vi "test_toml_reader.vi"(8 "error in (no error)":errorcluster, 11 "dragon_file_path":path=path "C:/Projects/toml-edit-labview/lv_src/test.toml") -> ()   [LabVIEW 2020]
uses:
  Doc/Doc.lvclass
  Table/Table.lvclass
  Item/Item.lvclass
  Value/Value.lvclass
  InlineTable/InlineTable.lvclass
  Item/type--enum.ctl
  Value/value_type--enum.ctl
panel:
  out "Contains Item":bool[](array[boolean])
  out "item_types":T1[](array[typedef])
  out "values":string[](array[string])
  out "item_names 2":string[](array[string])
  out "inline_table_item_names":string[](array[string])
  out "value_types":T2[](array[typedef])
  out "item_types":T1[](array[typedef])
  out "item_names":string[](array[string])
  out "value_strings":string[](array[string])
  out "item_names":string[](array[string])
  out "item_types":T1[](array[typedef])
  out "integer_value":i64
  out "string_value":string
  out "value_type":T2
  out "item_type":T1
  out "tables":string[](array[string])
  out "error out":errorcluster
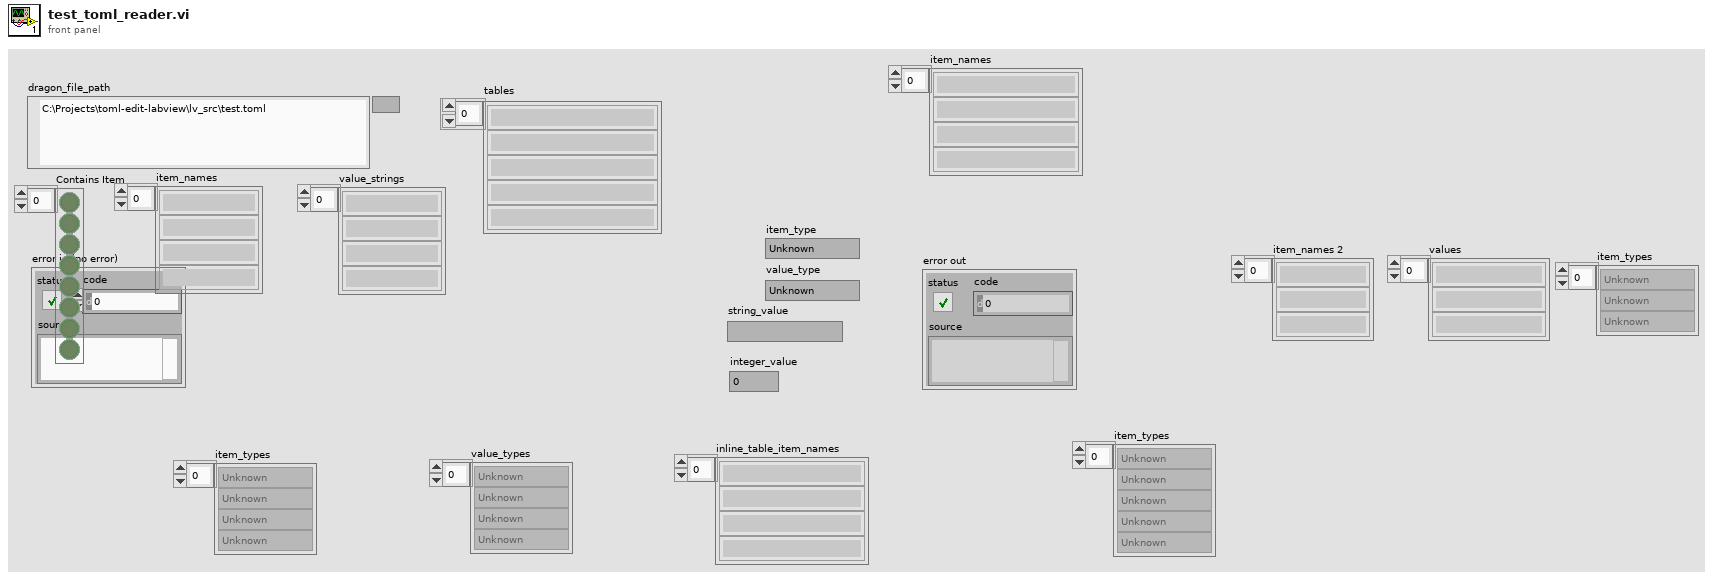
[diagram p1: front panel]
types:
  T1 = typedef "toml_edit.lvlib/Item.lvclass/type--enum.ctl" = enum16{"Unknown", "None", "Value", "ArrayOfTables", "Table"}
  T2 = typedef "toml_edit.lvlib/Value.lvclass/value_type--enum.ctl" = enum16{"Unknown", "String", "Integer", "Float", "Boolean", "Datetime", "Array", "InlineTable"}
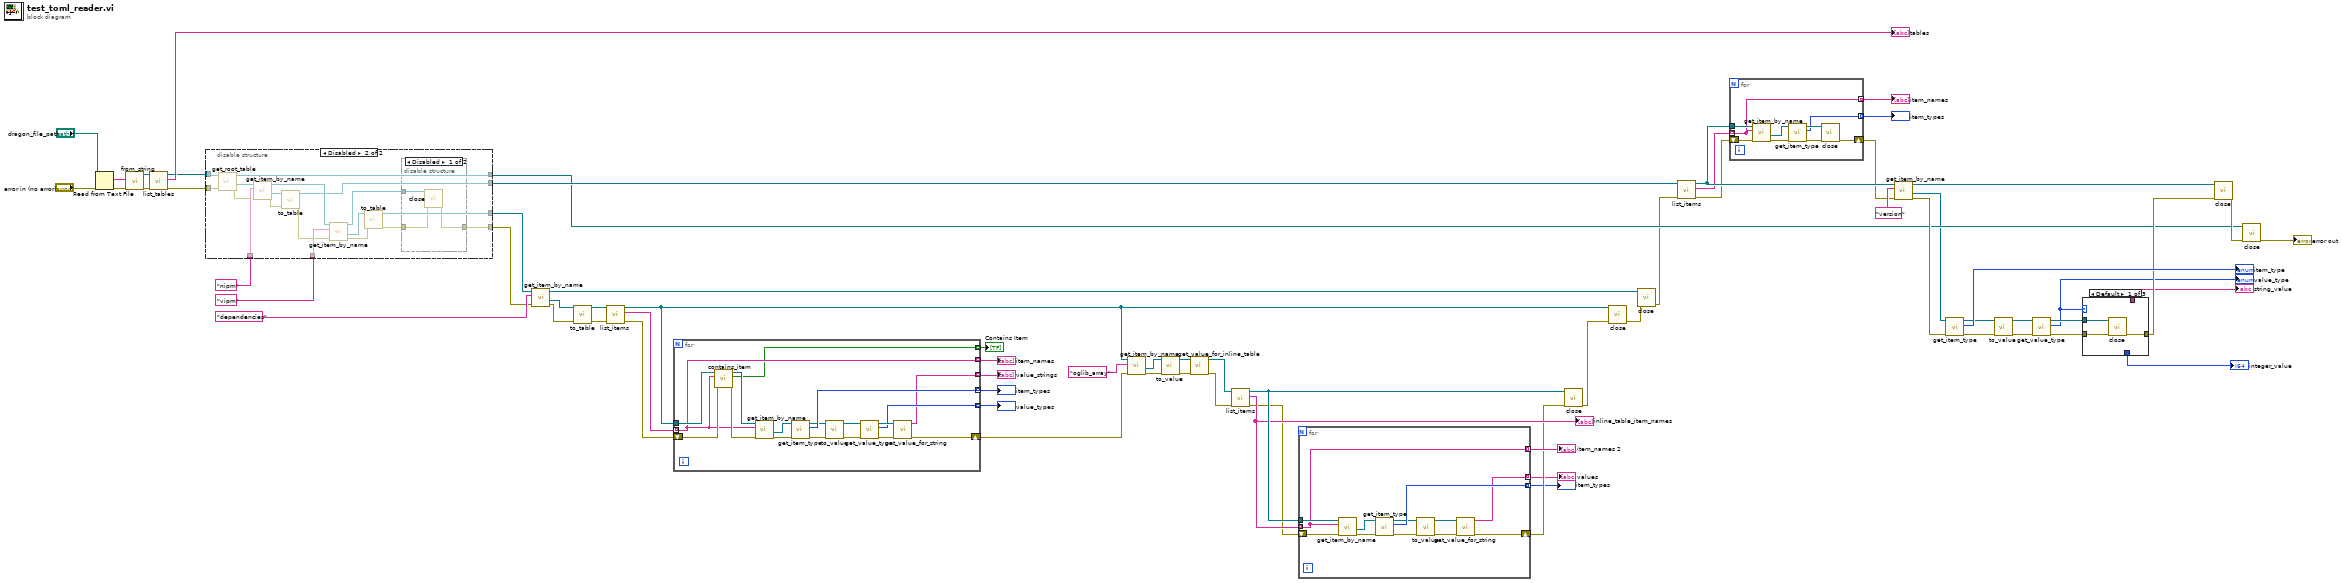
[diagram p0: block diagram]
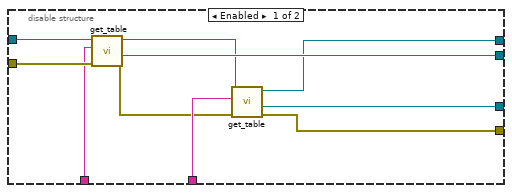
[diagram p2: hidden frame]
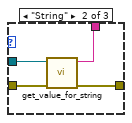
[diagram p4: hidden frame]
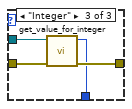
[diagram p5: hidden frame]
diagram:
  n1 = Read from Text File(file (use dialog)="dragon_file_path", error in="error in (no error)") -> (text=w67:string, error out=w66:errorcluster)  [unwired: 2 in, 2 out]
  n2 = call "from_string.vi"("error in (no error)"=w66, "toml"=w67) -> ("error out"=w64:errorcluster, "Doc out"=w65:refnum<class "Doc.lvclass">)  [unwired: 8 in]
  n3 = call "list_tables.vi"("error in (no error)"=w64, "Doc in"=w65) -> ("error out"=w61:errorcluster, "table_names"=→"tables":string[], "Doc out"=w62:refnum<class "Doc.lvclass">)  [unwired: 7 in]
  n4 = disable-structure shown="Disabled" {
    disable-tunnel: w62 -> [w80 w97]
    disable-tunnel: w61 -> [w79 w98]
    disable-tunnel: "nipm" ("table_name") -> [w78 w94]
    disable-tunnel: [w77 w90] -> w39
    disable-tunnel: [w75 w95] -> w38
    disable-tunnel: "vipm" ("table_name") -> [w74 w93]
    disable-tunnel: [w73 w88] -> w36
    disable-tunnel: [w72 w81] -> w19
    frame Enabled {
      n5 = call "get_table.vi"("error in (no error)"=w79, "table_name"=w78, "Doc in"=w80) -> ("error out"=w71:errorcluster, "Table"=w77:refnum<class "Table.lvclass">, "Doc out"=w76:refnum<class "Doc.lvclass">)  [unwired: 5 in, 1 out]
      n6 = call "get_table.vi"("error in (no error)"=w71, "table_name"=w74, "Doc in"=w76) -> ("error out"=w72:errorcluster, "Table"=w73:refnum<class "Table.lvclass">, "Doc out"=w75:refnum<class "Doc.lvclass">)  [unwired: 5 in, 1 out]
    }
    frame Disabled {
      n7 = call "get_root_table.vi"("error in (no error)"=w98, "Doc in"=w97) -> ("error out"=w84:errorcluster, "Table"=w96:refnum<class "Table.lvclass">, "Doc out"=w95:refnum<class "Doc.lvclass">)  [unwired: 7 in]
      n8 = call "get_item_by_name.vi"("error in (no error)"=w84, "item_name"=w94, "Table in"=w96) -> ("error out"=w85:errorcluster, "Item"=w91:refnum<class "Item.lvclass">, "Table out"=w92:refnum<class "Table.lvclass">)  [unwired: 4 in, 2 out]
      n9 = call "to_table.vi"("error in (no error)"=w85, "Item in"=w91) -> ("error out"=w86:errorcluster, "Table"=w90:refnum<class "Table.lvclass">)  [unwired: 8 in]
      n10 = call "get_item_by_name.vi"("error in (no error)"=w86, "item_name"=w93, "Table in"=w92) -> ("error out"=w87:errorcluster, "Item"=w89:refnum<class "Item.lvclass">, "Table out"=w83:refnum<class "Table.lvclass">)  [unwired: 4 in, 2 out]
      n11 = call "to_table.vi"("error in (no error)"=w87, "Item in"=w89) -> ("error out"=w82:errorcluster, "Table"=w88:refnum<class "Table.lvclass">)  [unwired: 8 in]
      n12 = disable-structure shown="Disabled" {
        disable-tunnel: w83 -> [w101 _]
        disable-tunnel: w82 -> [w100 w102]
        disable-tunnel: [w99 w102] -> w81
        frame Disabled {
          n13 = call "close.vi"("error in (no error)"=w100, "Table in"=w101) -> ("error out"=w99:errorcluster)  [unwired: 9 in]
        }
        frame Enabled {
        }
      }
    }
  }
  n14 = call "get_item_by_name.vi"("error in (no error)"=w19, "item_name"="dependencies" ("table_name"), "Table in"=w36) -> ("error out"=w33:errorcluster, "Item"=w18:refnum<class "Item.lvclass">, "Table out"=w31:refnum<class "Table.lvclass">)  [unwired: 4 in, 2 out]
  n15 = call "to_table.vi"("error in (no error)"=w33, "Item in"=w18) -> ("error out"=w34:errorcluster, "Table"=w21:refnum<class "Table.lvclass">)  [unwired: 8 in]
  n16 = call "list_items.vi"("error in (no error)"=w34, "Table in"=w21) -> ("error out"=w28:errorcluster, "items"=w29:string[], "Table out"=w23:refnum<class "Table.lvclass">)  [unwired: 7 in]
  n17 = for {
    tunnel: w23 -> [w108]
    tunnel: w29 -> [w105] mode=indexing
    shift-right: [w116] -> w22
    shift-left: w28 -> [w107]
    tunnel: [w119] -> w25 mode=indexing
    tunnel: [w105] -> w26 mode=indexing
    tunnel: [w103] -> w27 mode=indexing
    tunnel: [w112] -> w24 mode=indexing
    tunnel: [w104] -> w2 mode=indexing
    n18 = call "contains_item.vi"("error in (no error)"=w107, "item_name"=w105, "Table in"=w108) -> ("error out"=w106:errorcluster, "contains_item"=w104:bool, "Table out"=w109:refnum<class "Table.lvclass">)  [unwired: 6 in]
    n19 = call "get_item_by_name.vi"("error in (no error)"=w106, "item_name"=w105, "Table in"=w109) -> ("error out"=w120:errorcluster, "Item"=w110:refnum<class "Item.lvclass">)  [unwired: 4 in, 3 out]
    n20 = call "get_item_type.vi"("error in (no error)"=w120, "Item in"=w110) -> ("error out"=w117:errorcluster, "item_type"=w119:T1, "Item out"=w118:refnum<class "Item.lvclass">)  [unwired: 7 in]
    n21 = call "to_value.vi"("error in (no error)"=w117, "Item in"=w118) -> ("error out"=w114:errorcluster, "Value out"=w111:refnum<class "Value.lvclass">)  [unwired: 8 in]
    n22 = call "get_value_type.vi"("error in (no error)"=w114, "Value in"=w111) -> ("error out"=w113:errorcluster, "value_type"=w112:T2, "Value out"=w115:refnum<class "Value.lvclass">)  [unwired: 7 in]
    n23 = call "get_value_for_string.vi"("error in (no error)"=w113, "Value in"=w115) -> ("error out"=w116:errorcluster, "string_value"=w103:string)  [unwired: 8 in]
  }
  "value_strings" <- w27
  "item_names" <- w26
  "item_types" <- w25
  "value_types" <- w24
  "Contains Item" <- w2
  n24 = call "get_item_by_name.vi"("error in (no error)"=w22, "item_name"="oglib_array", "Table in"=w23) -> ("error out"=w15:errorcluster, "Item"=w3:refnum<class "Item.lvclass">)  [unwired: 4 in, 3 out]
  n25 = call "to_value.vi"("error in (no error)"=w15, "Item in"=w3) -> ("error out"=w14:errorcluster, "Value out"=w13:refnum<class "Value.lvclass">)  [unwired: 8 in]
  n26 = call "get_value_for_inline_table.vi"("error in (no error)"=w14, "Value in"=w13) -> ("error out"=w12:errorcluster, "InlineTable out"=w1:refnum<class "InlineTable.lvclass">)  [unwired: 8 in]
  n27 = call "list_items.vi"("error in (no error)"=w12, "Table in"=w1) -> ("error out"=w7:errorcluster, "items"=w8:string[], "Table out"=w9:refnum<class "InlineTable.lvclass">)  [unwired: 7 in]
  "inline_table_item_names" <- w8
  n28 = for {
    tunnel: w9 -> [w132]
    tunnel: w8 -> [w130] mode=indexing
    shift-right: [w128] -> w6
    shift-left: w7 -> [w131]
    tunnel: [w130] -> w10 mode=indexing
    tunnel: [w121] -> w5 mode=indexing
    tunnel: [w129] -> w4 mode=indexing
    n29 = call "get_item_by_name.vi"("error in (no error)"=w131, "key_name"=w130, "Table in"=w132) -> ("error out"=w127:errorcluster, "Item"=w122:refnum<class "Item.lvclass">)  [unwired: 6 in, 1 out]
    n30 = call "get_item_type.vi"("error in (no error)"=w127, "Item in"=w122) -> ("error out"=w126:errorcluster, "item_type"=w129:T1, "Item out"=w124:refnum<class "Item.lvclass">)  [unwired: 7 in]
    n31 = call "to_value.vi"("error in (no error)"=w126, "Item in"=w124) -> ("error out"=w125:errorcluster, "Value out"=w123:refnum<class "Value.lvclass">)  [unwired: 8 in]
    n32 = call "get_value_for_string.vi"("error in (no error)"=w125, "Value in"=w123) -> ("error out"=w128:errorcluster, "string_value"=w121:string)  [unwired: 8 in]
  }
  "item_names 2" <- w10
  "values" <- w5
  "item_types" <- w4
  n33 = call "close.vi"("error in (no error)"=w6, "Table in"=w9) -> ("error out"=w11:errorcluster)  [unwired: 9 in]
  n34 = call "close.vi"("error in (no error)"=w11, "Table in"=w23) -> ("error out"=w32:errorcluster)  [unwired: 9 in]
  n35 = call "close.vi"("error in (no error)"=w32, "Table in"=w31) -> ("error out"=w30:errorcluster)  [unwired: 9 in]
  n36 = call "list_items.vi"("error in (no error)"=w30, "Table in"=w39) -> ("error out"=w42:errorcluster, "items"=w44:string[], "Table out"=w45:refnum<class "Table.lvclass">)  [unwired: 7 in]
  n37 = for {
    tunnel: w45 -> [w141]
    tunnel: w44 -> [w134] mode=indexing
    shift-right: [w136] -> w41
    shift-left: w42 -> [w140]
    tunnel: [w135] -> w43 mode=indexing
    tunnel: [w134] -> w40 mode=indexing
    n38 = call "get_item_by_name.vi"("error in (no error)"=w140, "item_name"=w134, "Table in"=w141) -> ("error out"=w139:errorcluster, "Item"=w133:refnum<class "Item.lvclass">)  [unwired: 4 in, 3 out]
    n39 = call "get_item_type.vi"("error in (no error)"=w139, "Item in"=w133) -> ("error out"=w137:errorcluster, "item_type"=w135:T1, "Item out"=w138:refnum<class "Item.lvclass">)  [unwired: 7 in]
    n40 = call "close.vi"("error in (no error)"=w137, "Item in"=w138) -> ("error out"=w136:errorcluster)  [unwired: 9 in]
  }
  "item_types" <- w43
  "item_names" <- w40
  n41 = call "get_item_by_name.vi"("error in (no error)"=w41, "item_name"="version", "Table in"=w45) -> ("error out"=w58:errorcluster, "Item"=w17:refnum<class "Item.lvclass">, "Table out"=w56:refnum<class "Table.lvclass">)  [unwired: 4 in, 2 out]
  n42 = call "get_item_type.vi"("error in (no error)"=w58, "Item in"=w17) -> ("error out"=w53:errorcluster, "item_type"=→"item_type":T1, "Item out"=w54:refnum<class "Item.lvclass">)  [unwired: 7 in]
  n43 = call "to_value.vi"("error in (no error)"=w53, "Item in"=w54) -> ("error out"=w52:errorcluster, "Value out"=w20:refnum<class "Value.lvclass">)  [unwired: 8 in]
  n44 = call "get_value_type.vi"("error in (no error)"=w52, "Value in"=w20) -> ("error out"=w49:errorcluster, "value_type"=w47:T2, "Value out"=w50:refnum<class "Value.lvclass">)  [unwired: 7 in]
  "value_type" <- w47
  n45 = case shown="Default" w47 {
    tunnel: w50 -> [w144 w148 w152]
    tunnel: w49 -> [w142 w147 w151]
    tunnel: [w143 w146 w150] -> w51
    tunnel: [_ w145 _] -> w48
    tunnel: [_ _ w149] -> w46
    frame Default {
      n46 = call "close.vi"("error in (no error)"=w142, "Value in"=w144) -> ("error out"=w143:errorcluster)  [unwired: 9 in]
    }
    frame "String" {
      n47 = call "get_value_for_string.vi"("error in (no error)"=w147, "Value in"=w148) -> ("error out"=w146:errorcluster, "string_value"=w145:string)  [unwired: 8 in]
    }
    frame "Integer" {
      n48 = call "get_value_for_integer.vi"("error in (no error)"=w151, "Value in"=w152) -> ("error out"=w150:errorcluster, "integer_value"=w149:i64)  [unwired: 8 in]
    }
  }
  "string_value" <- w48
  "integer_value" <- w46
  n49 = call "close.vi"("error in (no error)"=w51, "Table in"=w56) -> ("error out"=w59:errorcluster)  [unwired: 9 in]
  n50 = call "close.vi"("error in (no error)"=w59, "Doc in"=w38) -> ("error out"=→"error out":errorcluster)  [unwired: 9 in]
